vi "Test Initialize Stores.vi"(8 "error in":errorcluster, 10 "Work Folder":path, 11 "Test Data Folder":path) -> (0 "error out":errorcluster, 2 "Report":string, 3 "Passed":bool)   [LabVIEW 2026]
doc: "Tests Initialize Stores.vi. On a copy of the version-1 test data (Test Data\\v1) it must migrate the folder to schema version 2 and open both stores. The v1 sample does hold one entry with End Time 0, in 2025-07, but Get Running Entry only looks at the current and the previous UTC month, so no entry is running. On a copy of the schema-v2 samples it must open the stores without migrating. Checks: Projects.ini carries Schema Version = 2 after the call; no running entry and an empty Running Entry ID; the migrated projects were read (TimeTracker is in the project list); the v2 samples open without error and list TimeTracker and Client Website.\n\nInputs: Test Data Folder; Work Folder; error in. Outputs: Passed; Report; error out.\n\nGenerated by: Claude"
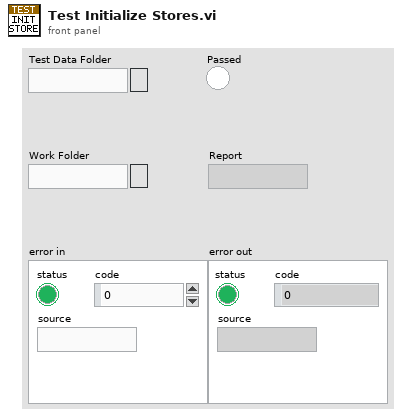
[diagram p1: front panel]
types:
  T1 = typedef "Time Entry.ctl" = cluster{"ID":string, "Project ID":string, "Task ID":string, "Start Time":timestamp, "End Time":timestamp, "Description":string}
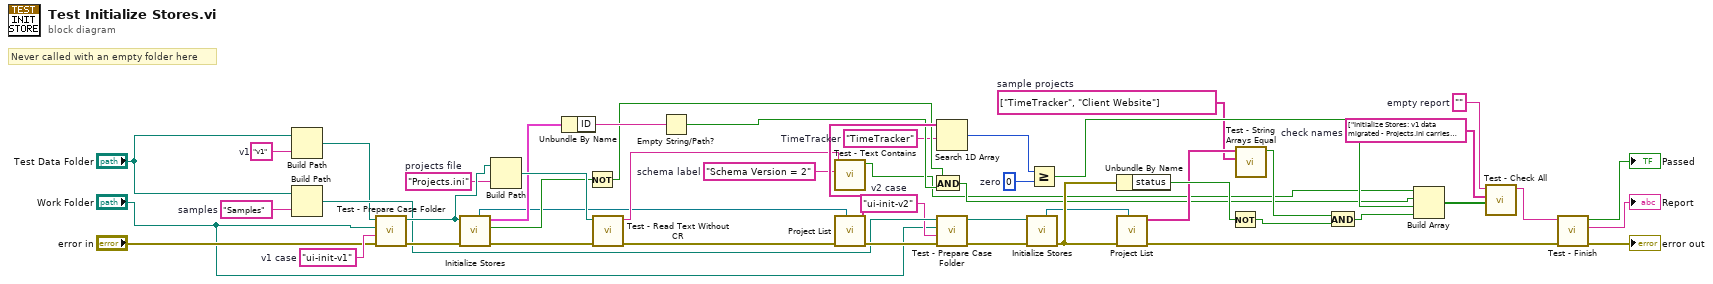
[diagram p0: block diagram]
diagram:
  w17 = string[] ["Initialize Stores: v1 data migrated - Projects.ini carries Schema Version = 2", "Initialize Stores: v1 data - no running entry and an empty Running Entry ID", "Initialize Stores: migrated projects were read (TimeTracker listed)", "Initialize Stores: v2 samples open without error and list their active projects"]  # check names
  w16 = string[] ["TimeTracker", "Client Website"]  # sample projects
  w15 = 0  # zero
  w14 = "TimeTracker"  # TimeTracker
  w13 = "Schema Version = 2"  # schema label
  w12 = "Projects.ini"  # projects file
  w11 = ""  # empty report
  w10 = "ui-init-v2"  # v2 case
  w9 = "ui-init-v1"  # v1 case
  w8 = "Samples"  # samples
  w7 = "v1"  # v1
  # "Never called with an empty folder here"
  n1 = Build Path(base path="Test Data Folder", name or relative path=w7) -> (appended path=w18:path)
  n2 = Build Path(base path="Test Data Folder", name or relative path=w8) -> (appended path=w19:path)
  n3 = call "Test - Prepare Case Folder.vi"("error in (no error)"="error in", "Case Name"=w9, "Work Folder"="Work Folder", "Source Folder"=w18) -> ("error out"=w21:errorcluster, "Case Folder"=w20:path)  [unwired: 6 in]
  n4 = call "Initialize Stores.vi"("error in"=w21, "Data Folder"=w20) -> ("error out"=w25:errorcluster, "Entry Running?"=w24:bool, "Running Entry"=w23:T1, "Project Store out"=w22:refnum<class "Project Store.lvclass">)  [unwired: 5 in, 1 out]
  n5 = Build Path(base path=w20, name or relative path=w12) -> (appended path=w26:path)
  n6 = Unbundle By Name(w23) -> ("ID"=w31:string)
  n7 = Not(x=w24) -> (.not. x?=w30:bool)
  n8 = call "Test - Read Text Without CR.vi"("error in (no error)"=w25, "File"=w26) -> ("error out"=w28:errorcluster, "Text"=w27:string)  [unwired: 8 in]
  n9 = Empty String/Path?(string/path=w31) -> (empty?=w32:bool)
  n10 = call "Test - Text Contains.vi"("Search Text"=w13, "Text"=w27) -> ("Contains?"=w29:bool)  [unwired: 8 in, 1 out]
  n11 = call "Project List.vi"("Project Store in"=w22, "error in"=w28) -> ("error out"=w35:errorcluster, "Project Names"=w34:string[])  [unwired: 6 in, 2 out]
  n12 = And(x=w30, y=w32) -> (x .and. y?=w33:bool)
  n13 = Search 1D Array(1D array=w34, element=w14) -> (index of element=w36:i32)  [unwired: 1 in]
  n14 = call "Test - Prepare Case Folder.vi"("error in (no error)"=w35, "Case Name"=w10, "Work Folder"="Work Folder", "Source Folder"=w19) -> ("error out"=w39:errorcluster, "Case Folder"=w38:path)  [unwired: 6 in]
  n15 = call "Initialize Stores.vi"("error in"=w39, "Data Folder"=w38) -> ("error out"=w41:errorcluster, "Project Store out"=w40:refnum<class "Project Store.lvclass">)  [unwired: 5 in, 3 out]
  n16 = Greater Or Equal?(x=w36, y=w15) -> (x >= y?=w37:bool)
  n17 = Unbundle By Name(w41) -> ("status"=w45:bool)
  n18 = call "Project List.vi"("Project Store in"=w40, "error in"=w41) -> ("error out"=w43:errorcluster, "Project Names"=w42:string[])  [unwired: 6 in, 2 out]
  n19 = Not(x=w45) -> (.not. x?=w46:bool)
  n20 = call "Test - String Arrays Equal.vi"("Expected"=w16, "Actual"=w42) -> ("Equal?"=w44:bool)  [unwired: 8 in, 1 out]
  n21 = And(x=w44, y=w46) -> (x .and. y?=w47:bool)
  n22 = Build Array(w29, w33, w37, w47) -> (w48:bool[])
  n23 = call "Test - Check All.vi"("Conditions"=w48, "Check Names"=w17, "Report in"=w11) -> ("Report out"=w49:string)  [unwired: 7 in, 1 out]
  n24 = call "Test - Finish.vi"("error in (no error)"=w43, "Report"=w49) -> ("error out"=→"error out":errorcluster, "Report out"=→"Report":string, "Passed"=→"Passed":bool)  [unwired: 7 in]
